vi "Pi_Variable.vi"(11 "Numeric":i32) -> ()   [LabVIEW 2024]
uses:
  <vilib>/Utility/error.llb/DialogTypeEnum.ctl
panel:
  out "x+y":dbl
  out "output array":T1(array[cluster])
  in  "Instructions":T1(array[cluster])=[{"Instruct Data"=0, "Op Code"=0, "Flags"=[FALSE, TRUE, TRUE, FALSE, FALSE, FALSE, FALSE, FALSE, FALSE, FALSE, FALSE, FALSE, FALSE, FALSE, FALSE, FALSE, FALSE, FALSE, FALSE, FALSE, FALSE, FALSE, FALSE, TRUE], "Comments"="0 Green", "Time (s)"=2e-06}, {"Instruct Data"=0, "Op Code"=0, "Flags"=[FALSE, FALSE, FALSE, FALSE, FALSE, FALSE, FALSE, FALSE, FALSE, FALSE, FALSE, FALSE, FALSE, FALSE, FALSE, FALSE, FALSE, FALSE, FALSE, FALSE, FALSE, FALSE, FALSE, FALSE], "Comments"="1", "Time (s)"=5e-07}, {"Instruct Data"=0, "Op Code"=0, "Flags"=[TRUE, TRUE, FALSE, FALSE, FALSE, FALSE, FALSE, FALSE, FALSE, FALSE, FALSE, FALSE, FALSE, FALSE, FALSE, FALSE, FALSE, FALSE, FALSE, FALSE, FALSE, FALSE, FALSE, FALSE], "Comments"="2", "Time (s)"=2.32e-07}, {"Instruct Data"=0, "Op Code"=6, "Flags"=[FALSE, TRUE, FALSE, FALSE, FALSE, FALSE, FALSE, FALSE, FALSE, FALSE, FALSE, FALSE, FALSE, FALSE, FALSE, FALSE, FALSE, FALSE, FALSE, FALSE, FALSE, FALSE, FALSE, FALSE], "Comments"="3", "Time (s)"=2e-06}, {"Instruct Data"=0, "Op Code"=0, "Flags"=[TRUE, FALSE, FALSE, FALSE, FALSE, FALSE, FALSE, FALSE, FALSE, FALSE, FALSE, FALSE, FALSE, FALSE, FALSE, FALSE, FALSE, FALSE, FALSE, FALSE, FALSE, FALSE, FALSE, FALSE], "Comments"="4", "Time (s)"=1.66e-07}, {"Instruct Data"=0, "Op Code"=0, "Flags"=[FALSE, TRUE, TRUE, FALSE, FALSE, FALSE, FALSE, FALSE, FALSE, FALSE, FALSE, FALSE, FALSE, FALSE, FALSE, FALSE, FALSE, FALSE, FALSE, FALSE, FALSE, FALSE, FALSE, FALSE], "Comments"="5", "Time (s)"=1e-07}, {"Instruct Data"=0, "Op Code"=6, "Flags"=[FALSE, TRUE, FALSE, FALSE, FALSE, FALSE, FALSE, FALSE, FALSE, FALSE, FALSE, FALSE, FALSE, FALSE, FALSE, FALSE, FALSE, FALSE, FALSE, FALSE, FALSE, FALSE, FALSE, FALSE], "Comments"="6", "Time (s)"=4.9e-06}, {"Instruct Data"=0, "Op Code"=6, "Flags"=[FALSE, FALSE, FALSE, FALSE, FALSE, FALSE, FALSE, FALSE, FALSE, FALSE, FALSE, FALSE, FALSE, FALSE, FALSE, FALSE, FALSE, FALSE, FALSE, FALSE, FALSE, FALSE, FALSE, FALSE], "Comments"="7", "Time (s)"=1e-06}, {"Instruct Data"=0, "Op Code"=0, "Flags"=[FALSE, FALSE, FALSE, FALSE, FALSE, FALSE, FALSE, FALSE, FALSE, FALSE, FALSE, FALSE, FALSE, FALSE, FALSE, FALSE, FALSE, FALSE, FALSE, FALSE, FALSE, FALSE, FALSE, FALSE], "Comments"="8", "Time (s)"=4e-07}, {"Instruct Data"=0, "Op Code"=0, "Flags"=[FALSE, TRUE, FALSE, FALSE, FALSE, FALSE, FALSE, FALSE, FALSE, FALSE, FALSE, FALSE, FALSE, FALSE, FALSE, FALSE, FALSE, FALSE, FALSE, FALSE, FALSE, FALSE, FALSE, FALSE], "Comments"="9", "Time (s)"=2e-06}, {"Instruct Data"=0, "Op Code"=0, "Flags"=[FALSE, TRUE, TRUE, FALSE, FALSE, FALSE, FALSE, FALSE, FALSE, FALSE, FALSE, FALSE, FALSE, FALSE, FALSE, FALSE, FALSE, FALSE, FALSE, FALSE, FALSE, FALSE, FALSE, FALSE], "Comments"="10", "Time (s)"=1e-07}, {"Instruct Data"=0, "Op Code"=0, "Flags"=[FALSE, TRUE, FALSE, FALSE, FALSE, FALSE, FALSE, FALSE, FALSE, FALSE, FALSE, FALSE, FALSE, FALSE, FALSE, FALSE, FALSE, FALSE, FALSE, FALSE, FALSE, FALSE, FALSE, FALSE], "Comments"="11", "Time (s)"=2.9e-06}, {"Instruct Data"=0, "Op Code"=6, "Flags"=[FALSE, FALSE, FALSE, FALSE, FALSE, FALSE, FALSE, FALSE, FALSE, FALSE, FALSE, FALSE, FALSE, FALSE, FALSE, FALSE, FALSE, FALSE, FALSE, FALSE, FALSE, FALSE, FALSE, FALSE], "Comments"="12", "Time (s)"=1e-06}] {"Time (s)" format="%.3p"; "Op Code" items=["Continue", "Stop", "Loop", "End Loop", "JSR", "RTS", "Branch", "Long Delay", "Wait"]}
  in  "Path to spinapi.dll":path=path "C:/SpinCore/SpinAPI/lib/spinapi.dll"
  in  "# of Instructions":u32=4
  in  "clock_freq (MHz)":dbl=500.0
  # "1) MW\n2) AOM\n3) SR400 Trigger"
  # "1"
  # "2"
  # "3"
  # "4"
  # "5"
  # "6"
  # "7"
  # "8"
  # "9"
  # "10"
  # "11"
  # "12"
  # "13"
  # "14"
  # "15"
  # "16"
  # "17"
  # "18"
  # "19"
  # "20"
  # "21"
  # "22"
  # "23"
  # "24"
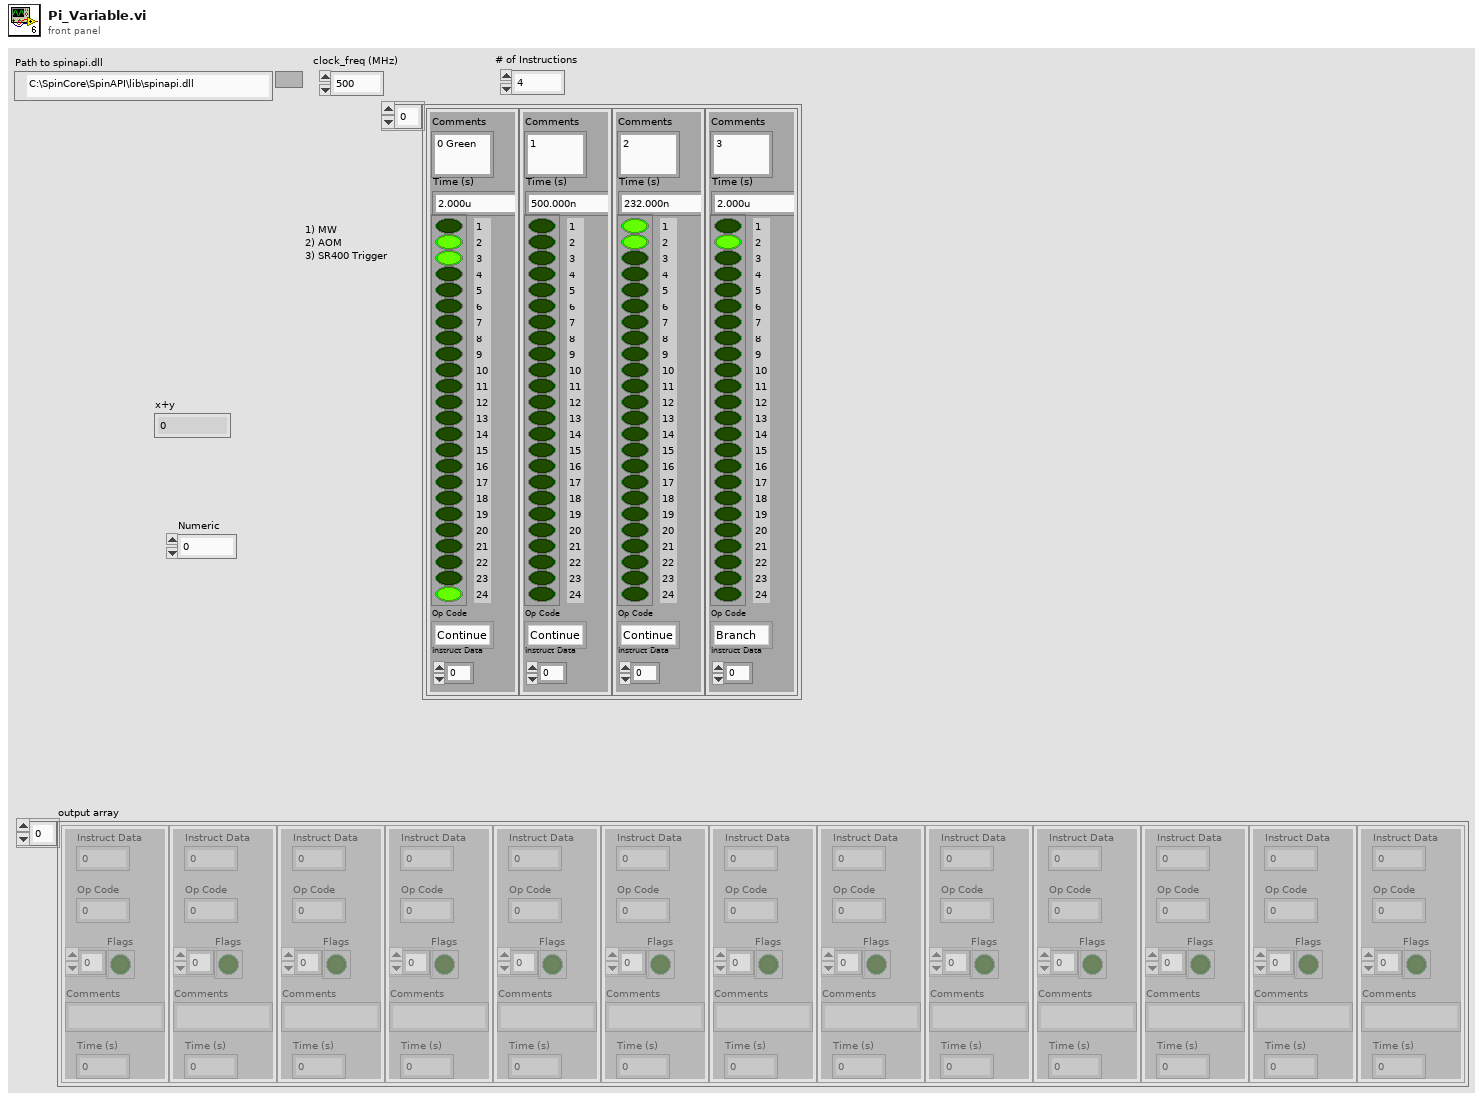
[diagram p1: front panel]
types:
  T1 = cluster{"Instruct Data":i32, "Op Code":i32, "Flags":bool[], "Comments":string, "Time (s)":dbl}[]
  T2 = typedef "DialogTypeEnum.ctl" = enum16{"no dialog", "OK message", "continue or stop message", "auto error handling dialog", "OK message + warnings", "continue/stop + warnings"}
  T3 = enum16{"Pulse Program", "Frequency Registers", "TX Phase Registers", "RX Phase Registers"}
  T4 = cluster{"Instruct Data":i32, "Op Code":i32, "Flags":bool[], "Comments":string, "Time (s)":dbl}
  T5 = cluster{"Instruct Data":i32, "Op Code":i32, "Flags":bool[], "Comments":string, dbl}
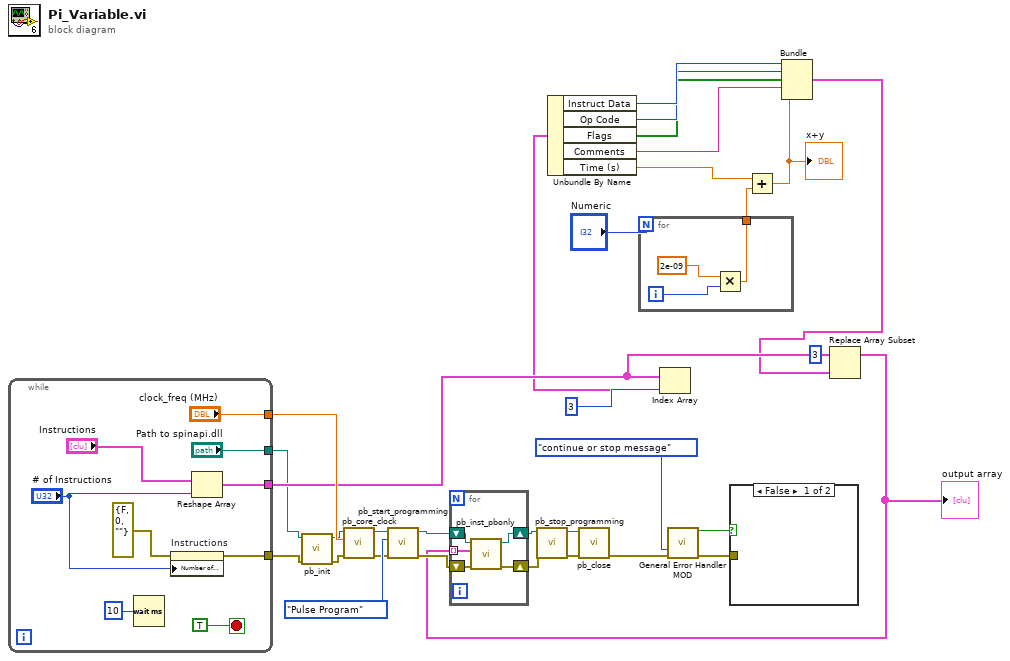
[diagram p0: block diagram]
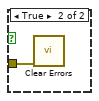
[diagram p2: hidden frame]
diagram:
  n1 = while {
    tunnel: [w38] -> w4
    tunnel: [w39] -> w11
    tunnel: ["Path to spinapi.dll"] -> w5
    tunnel: ["clock_freq (MHz)"] -> w20
    stop <- TRUE ("load") stop-if-true
    n2 = Wait (ms)(milliseconds to wait=u32 10) -> ()  [unwired: 1 out]
    n3 = property on="Instructions" class="Arr (strict)"(error in=errorcluster {"status"=FALSE, "code"=0, "source"=""} ("error in (no error)"), "Number of Columns"="# of Instructions") -> (error out=w38:errorcluster)  [unwired: 1 in, 1 out]
    n4 = Reshape Array "Reshape Array"("Instructions", "# of Instructions") -> (w39:T1)
  }
  n5 = call "pb_init.vi"("error in (no error)"=w4, "path in"=w5) -> ("error out"=w3:errorcluster, "path out"=w2:path)  [unwired: 8 in]
  n6 = call "pb_core_clock.vi"("error in (no error)"=w3, "clock_freq (MHz)"=w20, "path in"=w2) -> ("error out"=w21:errorcluster, "path out"=w22:path)  [unwired: 7 in]
  n7 = call "pb_start_programming.vi"("error in (no error)"=w21, "Device"=T3."Pulse Program", "path in"=w22) -> ("error out"=w28:errorcluster, "path out"=w32:path)  [unwired: 1 in, 6 out]
  n8 = for {
    N: "Numeric" -> [_]
    tunnel: [w42] -> w7
    i -> [w43]
    n9 = Multiply(x=2e-09, y=w43) -> (x*y=w42:dbl)
  }
  n10 = Index Array "Index Array"(array=w11, index=3) -> (element=w10:T4)
  n11 = Unbundle By Name "Unbundle By Name"(w10) -> ("Instruct Data"=w17:i32, "Op Code"=w16:i32, "Flags"=w15:bool[], "Comments"=w14:string, "Time (s)"=w13:dbl)
  n12 = Add(x=w13, y=w7) -> (x+y=w12:dbl)
  "x+y" <- w12
  n13 = Bundle("Instruct Data"=w17, "Op Code"=w16, "Flags"=w15, "Comments"=w14, w12) -> (w8:T5)  [unwired: 1 in]
  n14 = Replace Array Subset "Replace Array Subset"(array=w11, new element=w8, index=3) -> (w1:T1)
  "output array" <- w1
  n15 = for {
    tunnel: w1 -> [w46] mode=indexing
    shift-right: [w48] -> w30
    shift-left: w32 -> [w49]
    shift-right: [w45] -> w27
    shift-left: w28 -> [w47]
    n16 = call "pb_inst_pbonly.vi"("error in (no error)"=w47, "PB Instruction"=w46, "path in"=w49) -> ("error out"=w45:errorcluster, "path out"=w48:path)  [unwired: 2 in, 5 out]
  }
  n17 = call "pb_stop_programming.vi"("error in (no error)"=w27, "path in"=w30) -> ("error out"=w26:errorcluster, "path out"=w31:path)  [unwired: 1 in, 7 out]
  n18 = call "pb_close.vi"("error in (no error)"=w26, "path in"=w31) -> ("error out"=w19:errorcluster)  [unwired: 9 out]
  n19 = call "General Error Handler MOD.vi"("type of dialog (OK msg:1)"=DialogTypeEnum."continue or stop message", "error in (no error)"=w19) -> ("STOP?"=w23:bool, "error out"=w24:errorcluster)  [unwired: 12 out]
  n20 = case shown="False" w23 {
    tunnel: w24 -> [_ w50]
    frame False {
    }
    frame True {
      n21 = call <vilib>:"Clear Errors.vi"("error in (no error)"=w50) -> ()  [unwired: 1 in, 6 out]
    }
  }
